vi "ALL - VarMan VIs.vi"() -> ()   [LabVIEW 2021]
doc: "::: CalcExpress Toolkit :::\nCopyright (c) 2000-2026 Konstantin Shifershteyn. All rights reserved."
uses:
  cetypes.llb/VarMan Variable Context Handle.ctl
  cetypes.llb/VarMan Error Code.ctl
panel:
  in  "False":bool
  out "err code":T1 items=["No error", "Invalid variable type", "Variable not found", "Variable already exists", "Invalid context handle", "Input error", "Invalid data format", "No history attached", "History already attached", "Invalid history parameters", "Wrong variable name", "Wrong alias name", "Non-unique alias", "Alias not found", "No alias associated", "Alias already associated", "Wrong context name", "Non-unique context name", "Context name not found", "Invalid parameter", "Generic error", "Memory Full", "Unrecognized LV error", "Unknown error code"]
  in  "VC Handle":T2=-1
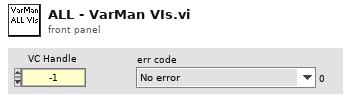
[diagram p1: front panel]
types:
  T1 = typedef "VarMan Error Code.ctl" = u16
  T2 = typedef "VarMan Variable Context Handle.ctl" = i32
  T3 = cluster{"datatype":u32, "STR":string, "DBL":dbl}[]
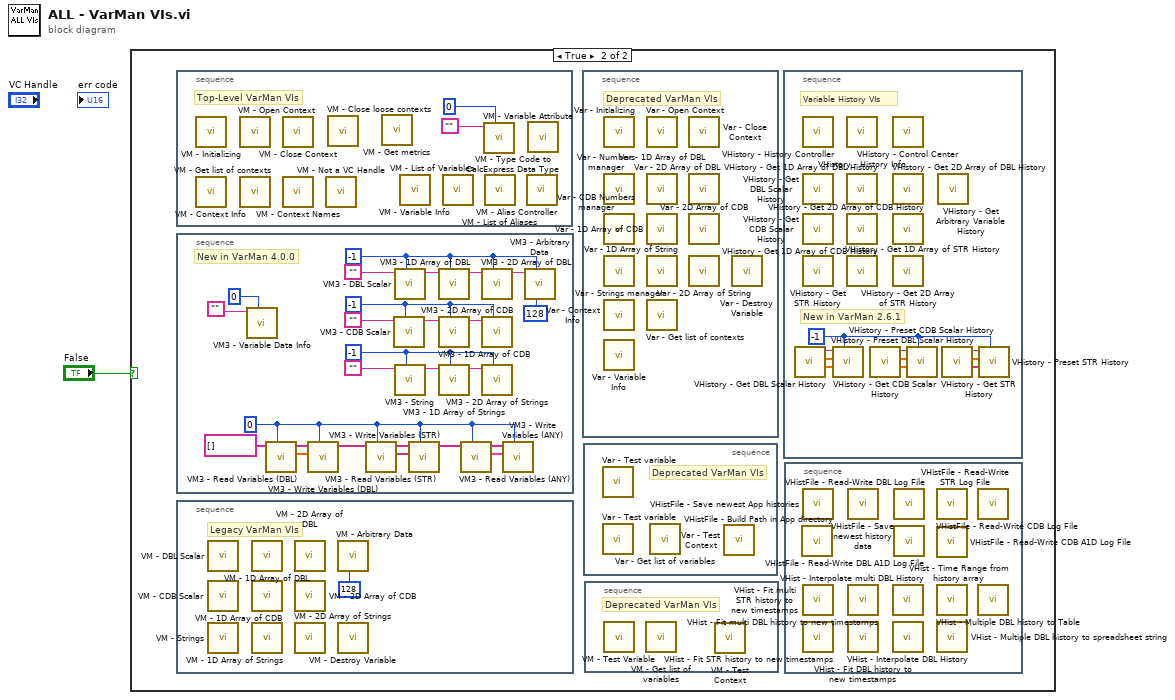
[diagram p0: block diagram]
diagram:
  n1 = case shown="True" "False" {
    frame False {
    }
    frame True {
      n2 = stacked-sequence {
        frame #0 {
          # "Top-Level VarMan VIs"
          n3 = call "VM - Initializing.vi"() -> ()  [unwired: 10 in, 2 out]
          n4 = call "VM - Context Info.vi"() -> ()  [unwired: 7 in, 5 out]
          n5 = call "VM - Open Context.vi"() -> ()  [unwired: 9 in, 3 out]
          n6 = call "VM - Get list of contexts.vi"() -> ()  [unwired: 7 in, 3 out]
          n7 = call "VM - Close Context.vi"() -> ()  [unwired: 10 in, 2 out]
          n8 = call "VM - Context Names.vi"() -> ()  [unwired: 6 in, 4 out]
          n9 = call "VM - Not a VC Handle.vi"() -> ()  [unwired: 2 in, 1 out]
          n10 = call "VM - Close loose contexts.vi"() -> ()  [unwired: 10 in, 2 out]
          n11 = call "VM - Get metrics.vi"() -> ()  [unwired: 7 in, 5 out]
          n12 = call "VM - Variable Info.vi"() -> ()  [unwired: 6 in, 6 out]
          n13 = call "VM - List of Variables.vi"() -> ()  [unwired: 7 in, 3 out]
          n14 = call "VM - Variable Attribute.vi"("VC Handle"=T2 0, "name_spec"="") -> ()  [unwired: 4 in, 6 out]
          n15 = call "VM - List of Aliases.vi"() -> ()  [unwired: 10 in, 2 out]
          n16 = call "VM - Alias Controller.vi"() -> ()  [unwired: 8 in, 4 out]
          n17 = call "VM - Type Code to CalcExpress Data Type.vi"() -> ()  [unwired: 11 in, 1 out]
        }
      }
      n18 = stacked-sequence {
        frame #0 {
          w7 = T2 -1 ("VC Handle")
          w2 = T2 -1 ("VC Handle")
          w9 = T2 -1 ("VC Handle")
          w21 = T2 0 ("VC Handle")
          # "New in VarMan 4.0.0"
          n19 = call "VM3 - Variable Data Info.vi"("VC Handle"=T2 0, "name_spec"="") -> ()  [unwired: 4 in, 6 out]
          n20 = call "VM3 - Read Variables (DBL).vi"("VC Handle"=w21, "name_specs"=string[] []) -> ("values out"=w25:dbl[], "dup name_specs"=w24:string[])  [unwired: 5 in, 3 out]
          n21 = call "VM3 - Write Variables (DBL).vi"("VC Handle"=w21, "values in"=w25, "name_specs"=w24) -> ("dup name_specs"=w22:string[])  [unwired: 5 in, 3 out]
          n22 = call "VM3 - Read Variables (STR).vi"("VC Handle"=w21, "name_specs"=w22) -> ("values out"=w19:string[], "dup name_specs"=w20:string[])  [unwired: 5 in, 3 out]
          n23 = call "VM3 - CDB Scalar.vi"("VC Handle"=w7, "name_spec"="") -> ("dup name_spec"=w6:string)  [unwired: 6 in, 3 out]
          n24 = call "VM3 - DBL Scalar.vi"("VC Handle"=w9, "name_spec"="") -> ("dup name_spec"=w11:string)  [unwired: 6 in, 3 out]
          n25 = call "VM3 - String.vi"("VC Handle"=w2, "name_spec"="") -> ("dup name_spec"=w4:string)  [unwired: 6 in, 3 out]
          n26 = call "VM3 - Write Variables (STR).vi"("VC Handle"=w21, "values in"=w19, "name_specs"=w20) -> ("dup name_specs"=w18:string[])  [unwired: 5 in, 3 out]
          n27 = call "VM3 - 1D Array of DBL.vi"("VC Handle"=w9, "name_spec"=w11) -> ("dup name_spec"=w8:string)  [unwired: 6 in, 3 out]
          n28 = call "VM3 - 1D Array of CDB.vi"("VC Handle"=w7, "name_spec"=w6) -> ("dup name_spec"=w5:string)  [unwired: 6 in, 3 out]
          n29 = call "VM3 - 1D Array of Strings.vi"("VC Handle"=w2, "name_spec"=w4) -> ("dup name_spec"=w3:string)  [unwired: 6 in, 3 out]
          n30 = call "VM3 - Read Variables (ANY).vi"("VC Handle"=w21, "name_specs"=w18) -> ("values out"=w27:T3, "dup name_specs"=w26:string[])  [unwired: 5 in, 3 out]
          n31 = call "VM3 - 2D Array of DBL.vi"("VC Handle"=w9, "name_spec"=w8) -> ("dup name_spec"=w10:string)  [unwired: 6 in, 3 out]
          n32 = call "VM3 - 2D Array of CDB.vi"("VC Handle"=w7, "name_spec"=w5) -> ()  [unwired: 6 in, 4 out]
          n33 = call "VM3 - 2D Array of Strings.vi"("VC Handle"=w2, "name_spec"=w3) -> ()  [unwired: 6 in, 4 out]
          n34 = call "VM3 - Write Variables (ANY).vi"("VC Handle"=w21, "values in"=w27, "name_specs"=w26) -> ()  [unwired: 5 in, 4 out]
          n35 = call "VM3 - Arbitrary Data.vi"("var type in"=u32 128 ("var type"), "VC Handle"=w9, "name_spec"=w10) -> ()  [unwired: 4 in, 5 out]
        }
      }
      n36 = stacked-sequence {
        frame #0 {
          # "Legacy VarMan VIs"
          n37 = call "VM - DBL Scalar.vi"() -> ()  [unwired: 6 in, 6 out]
          n38 = call "VM - CDB Scalar.vi"() -> ()  [unwired: 6 in, 6 out]
          n39 = call "VM - Strings.vi"() -> ()  [unwired: 6 in, 6 out]
          n40 = call "VM - 1D Array of DBL.vi"() -> ()  [unwired: 6 in, 6 out]
          n41 = call "VM - 1D Array of CDB.vi"() -> ()  [unwired: 6 in, 6 out]
          n42 = call "VM - 1D Array of Strings.vi"() -> ()  [unwired: 6 in, 6 out]
          n43 = call "VM - 2D Array of DBL.vi"() -> ()  [unwired: 6 in, 6 out]
          n44 = call "VM - 2D Array of CDB.vi"() -> ()  [unwired: 6 in, 6 out]
          n45 = call "VM - 2D Array of Strings.vi"() -> ()  [unwired: 6 in, 6 out]
          n46 = call "VM - Arbitrary Data.vi"("var type"=u32 128) -> ()  [unwired: 5 in, 6 out]
          n47 = call "VM - Destroy Variable.vi"() -> ()  [unwired: 8 in, 4 out]
        }
      }
      n48 = stacked-sequence {
        frame #0 {
          # "Deprecated VarMan VIs"
          n49 = call "Var - Initializing"() -> ()  [unwired: 10 in, 2 out]
          n50 = call "Var - Numbers manager"() -> ()  [unwired: 7 in, 5 out]
          n51 = call "Var - CDB Numbers manager"() -> ()  [unwired: 7 in, 5 out]
          n52 = call "Var - Strings manager"() -> ()  [unwired: 7 in, 5 out]
          n53 = call "Var - Context Info.vi"() -> ()  [unwired: 6 in, 6 out]
          n54 = call "Var - Variable Info.vi"() -> ()  [unwired: 5 in, 7 out]
          n55 = call "Var - Open Context"() -> ()  [unwired: 9 in, 3 out]
          n56 = call "Var - 1D Array of DBL"() -> ()  [unwired: 7 in, 5 out]
          n57 = call "Var - 1D Array of CDB"() -> ()  [unwired: 7 in, 5 out]
          n58 = call "Var - 1D Array of String"() -> ()  [unwired: 7 in, 5 out]
          n59 = call "Var - Get list of contexts"() -> ()  [unwired: 7 in, 3 out]
          n60 = call "Var - Close Context"() -> ()  [unwired: 10 in, 2 out]
          n61 = call "Var - 2D Array of DBL"() -> ()  [unwired: 7 in, 5 out]
          n62 = call "Var - 2D Array of CDB"() -> ()  [unwired: 7 in, 5 out]
          n63 = call "Var - 2D Array of String"() -> ()  [unwired: 7 in, 5 out]
          n64 = call "Var - Destroy Variable"() -> ()  [unwired: 8 in, 4 out]
        }
      }
      n65 = stacked-sequence {
        frame #0 {
          # "Deprecated VarMan VIs"
          n66 = call "Var - Test variable.vi"() -> ()  [unwired: 5 in, 5 out]
          n67 = call "Var - Test variable"() -> ()  [unwired: 5 in, 5 out]
          n68 = call "Var - Get list of variables"() -> ()  [unwired: 6 in, 4 out]
          n69 = call "Var - Test Context"() -> ()  [unwired: 9 in, 3 out]
        }
      }
      n70 = stacked-sequence {
        frame #0 {
          # "Deprecated VarMan VIs"
          n71 = call "VM - Test Variable.vi"() -> ()  [unwired: 5 in, 5 out]
          n72 = call "VM - Get list of variables.vi"() -> ()  [unwired: 6 in, 4 out]
          n73 = call "VM - Test Context.vi"() -> ()  [unwired: 9 in, 3 out]
        }
      }
      n74 = stacked-sequence {
        frame #0 {
          w29 = T2 -1 ("VC Handle")
          # "New in VarMan 2.6.1"
          # "Variable History VIs"
          n75 = call "VHistory - Get DBL Scalar History.vi"() -> ("history"=w37:dbl[], "time stamps"=w38:dbl[], "dup name_spec"=w36:string)  [unwired: 7 in, 2 out]
          n76 = call "VHistory - History Controller.vi"() -> ()  [unwired: 8 in, 4 out]
          n77 = call "VHistory - Get DBL Scalar History.vi"() -> ()  [unwired: 7 in, 5 out]
          n78 = call "VHistory - Get CDB Scalar History.vi"() -> ()  [unwired: 7 in, 5 out]
          n79 = call "VHistory - Get STR History.vi"() -> ()  [unwired: 7 in, 5 out]
          n80 = call "VHistory - Preset DBL Scalar History.vi"("VC Handle"=w29, "history"=w37, "time stamps"=w38, "name_spec"=w36) -> ()  [unwired: 6 in, 2 out]
          n81 = call "VHistory - History Info.vi"() -> ()  [unwired: 7 in, 5 out]
          n82 = call "VHistory - Get 1D Array of DBL History.vi"() -> ()  [unwired: 7 in, 5 out]
          n83 = call "VHistory - Get 1D Array of CDB History.vi"() -> ()  [unwired: 7 in, 5 out]
          n84 = call "VHistory - Get 1D Array of STR History.vi"() -> ()  [unwired: 7 in, 5 out]
          n85 = call "VHistory - Get CDB Scalar History.vi"() -> ("history"=w30:cdb[], "time stamps"=w31:dbl[], "dup name_spec"=w32:string)  [unwired: 7 in, 2 out]
          n86 = call "VHistory - Control Center.vi"() -> ()  [unwired: 9 in, 3 out]
          n87 = call "VHistory - Get 2D Array of DBL History.vi"() -> ()  [unwired: 7 in, 5 out]
          n88 = call "VHistory - Get 2D Array of CDB History.vi"() -> ()  [unwired: 7 in, 5 out]
          n89 = call "VHistory - Get 2D Array of STR History.vi"() -> ()  [unwired: 7 in, 5 out]
          n90 = call "VHistory - Preset CDB Scalar History.vi"("VC Handle"=w29, "history"=w30, "time stamps"=w31, "name_spec"=w32) -> ()  [unwired: 6 in, 2 out]
          n91 = call "VHistory - Get Arbitrary Variable History.vi"() -> ()  [unwired: 7 in, 5 out]
          n92 = call "VHistory - Get STR History.vi"() -> ("history"=w33:string[], "time stamps"=w34:dbl[], "dup name_spec"=w35:string)  [unwired: 7 in, 2 out]
          n93 = call "VHistory - Preset STR History.vi"("VC Handle"=w29, "history"=w33, "time stamps"=w34, "name_spec"=w35) -> ()  [unwired: 6 in, 2 out]
        }
      }
      n94 = stacked-sequence {
        frame #0 {
          n95 = call "VHistFile - Build Path in App directory.vi"() -> ()  [unwired: 5 in, 1 out]
          n96 = call "VHistFile - Save newest App histories.vi"() -> ()  [unwired: 11 in, 1 out]
          n97 = call "VHist - Fit multi STR history to new timestamps.vi"() -> ()  [unwired: 9 in, 3 out]
          n98 = call "VHist - Fit STR history to new timestamps.vi"() -> ()  [unwired: 9 in, 3 out]
          n99 = call "VHistFile - Save newest history data.vi"() -> ()  [unwired: 8 in, 4 out]
          n100 = call "VHist - Fit multi DBL history to new timestamps.vi"() -> ()  [unwired: 9 in, 3 out]
          n101 = call "VHist - Fit DBL history to new timestamps.vi"() -> ()  [unwired: 9 in, 3 out]
          n102 = call "VHist - Interpolate multi DBL History.vi"() -> ()  [unwired: 9 in, 3 out]
          n103 = call "VHist - Interpolate DBL History.vi"() -> ()  [unwired: 9 in, 3 out]
          n104 = call "VHistFile - Read-Write DBL Log File.vi"() -> ()  [unwired: 9 in, 3 out]
          n105 = call "VHistFile - Read-Write DBL A1D Log File.vi"() -> ()  [unwired: 9 in, 3 out]
          n106 = call "VHistFile - Read-Write CDB Log File.vi"() -> ()  [unwired: 9 in, 3 out]
          n107 = call "VHistFile - Read-Write CDB A1D Log File.vi"() -> ()  [unwired: 9 in, 3 out]
          n108 = call "VHist - Multiple DBL history to Table.vi"() -> ()  [unwired: 9 in, 3 out]
          n109 = call "VHist - Multiple DBL history to spreadsheet string.vi"() -> ()  [unwired: 10 in, 2 out]
          n110 = call "VHistFile - Read-Write STR Log File.vi"() -> ()  [unwired: 9 in, 3 out]
          n111 = call "VHist - Time Range from history array.vi"() -> ()  [unwired: 5 in, 2 out]
        }
      }
    }
  }
